vi "example test.vi"() -> (3 "correct execution settings":bool)   [LabVIEW 2015, in "tdms logger tests.lvlib"]
uses:
  tdms logger tests.lvlib
  execution/TDMS datalogger runtime.lvclass
  <vilib>/NI/Tag Bus/dictionary/data dictionary.lvclass/data dictionary.ctl
  <vilib>/NI/Tag Bus/dictionary/lookup polymorphs/locate double.vi
  <vilib>/NI/Tag Bus/table/data polymorphs/write one/write Double.vi
  <vilib>/NI/Tag Bus/dictionary/search/find data index.vi
  <vilib>/NI/Tag Bus/dictionary/search/search string list.vi
  <vilib>/NI/Tag Bus/dictionary/tag not found.vi
  configuration/TDMS datalogger configuration.lvclass
  <vilib>/NI/Tag Bus Module Framework/channel/TBM channel.lvclass
  <vilib>/NI/Tag Bus/tag/Data Type.ctl
  <vilib>/NI/Tag Bus/tag/tag descriptor.lvclass
  <vilib>/NI/Tag Bus Module Framework/channel/channel classification.ctl
  <vilib>/NI/Tag Bus/dictionary/data dictionary.lvclass
  <vilib>/NI/Tag Bus/table/data table.lvlib
  <vilib>/NI/Configuration Framework/serializable configuration/NISE_CEF_serializable configuration.lvclass
panel:
  out "final error":errorcluster
  out "output error":errorcluster
  out "output lookup error":errorcluster
  out "init error":errorcluster
  out "serialization problem":errorcluster
  out "invalid configuration":errorcluster
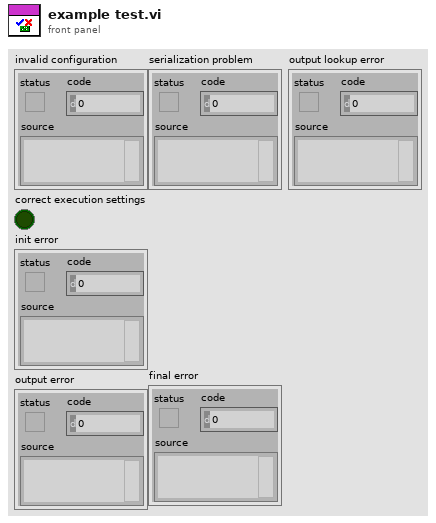
[diagram p1: front panel]
types:
  T1 = typedef "TBM channel.lvclass/channel classification.ctl" = enum16{"input data", "output data", "processing parameter", "processing result"}
  T2 = typedef "tag bus.lvlib/tag descriptor.lvclass/Data Type.ctl" = enum16{"Double", "Single", "I64", "I32", "I16", "I8", "U64", "U32", "U16", "U8", "Boolean", "String", "Array of Double", "Array of Single", "Array of I64", "Array of I32", "Array of I16", "Array of I8", "Array of U64", "Array of U32", "Array of U16", "Array of U8", "Array of Boolean", "Array of String"}
  T3 = typedef "TBM channel.lvclass/data tables.ctl" = cluster{"input data":T4, "processing parameter":T4, "processing result":T4, "output data":T4}
  T4 = typedef "tag bus.lvlib/dictionary table pair.ctl" = cluster{"data dictionary":refnum<class "data dictionary.lvclass">, "data table":T5}
  T5 = typedef "tag bus.lvlib/data table.lvlib/data table.ctl" = cluster{"Double":dbl[], "Single":sgl[], "I64":i64[], "I32":i32[], "I16":i16[], "I8":i8[], "U64":u64[], "U32":u32[], "U16":u16[], "U8":u8[], "Boolean":bool[], "String":string[], "Array of Double":cluster{"DBL Array":dbl[]}[], "Array of Single":cluster{"SGL Array":sgl[]}[], "Array of I64":cluster{"I64 Array":i64[]}[], "Array of I32":cluster{"I32 Array":i32[]}[], "Array of I16":cluster{"I16 Array":i16[]}[], "Array of I8":cluster{"I8 Array":i8[]}[], "Array of U64":cluster{"U64 Array":u64[]}[], "Array of U32":cluster{"U32 Array":u32[]}[], "Array of U16":cluster{"U16 Array":u16[]}[], "Array of U8":cluster{"U8 Array":u8[]}[], "Array of Boolean":cluster{"Boolean Array":bool[]}[], "Array of String":cluster{"String Array":string[]}[]}
  T6 = typedef "TBM module execution interface.lvclass/execution settings.ctl" = cluster{"reads inputs":bool, "processes data":bool, "writes outputs":bool}
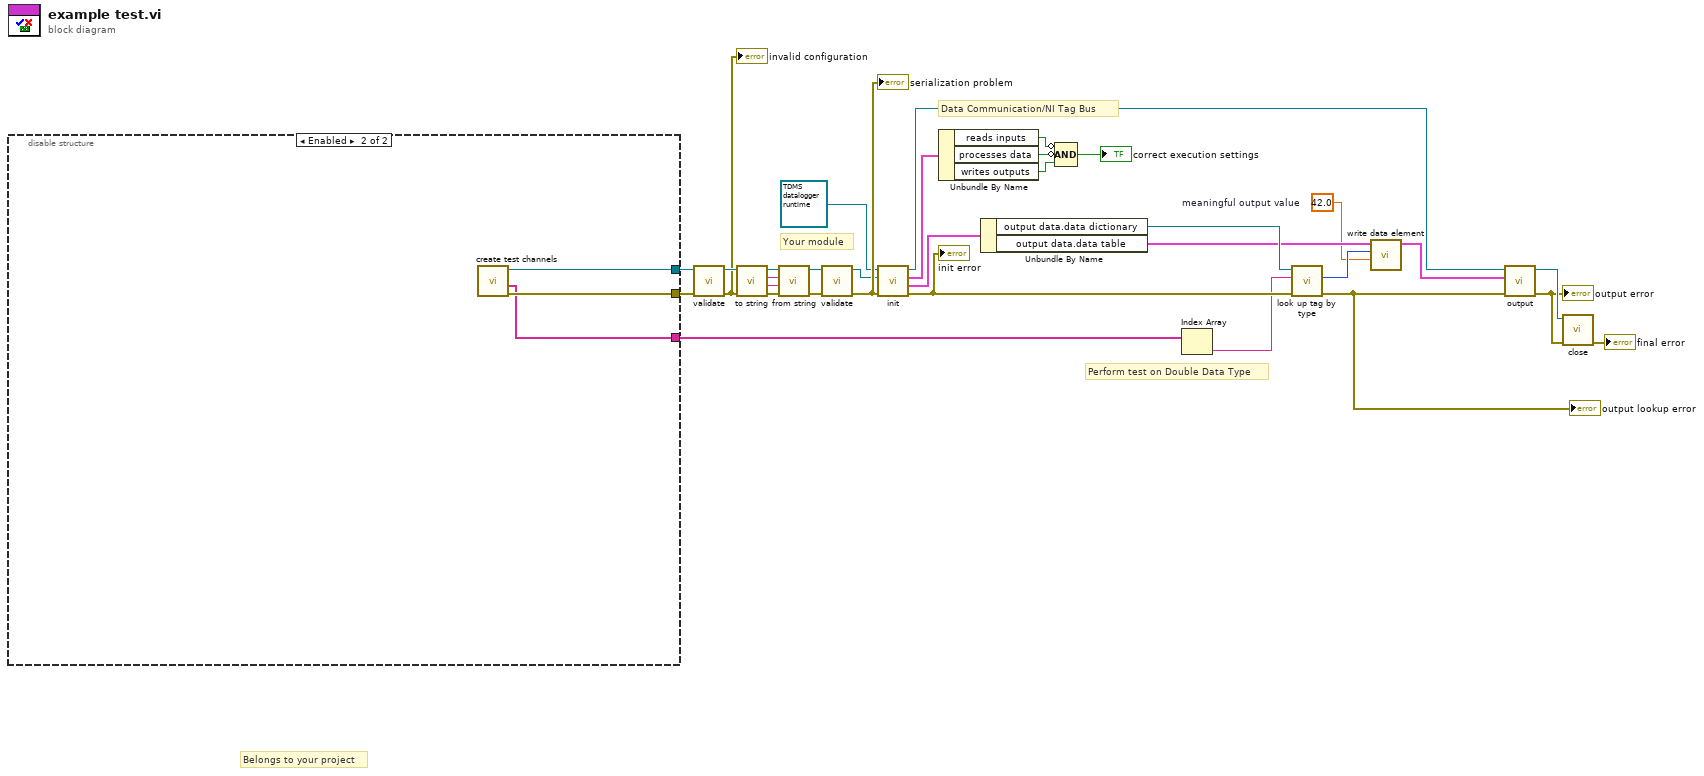
[diagram p0: block diagram]
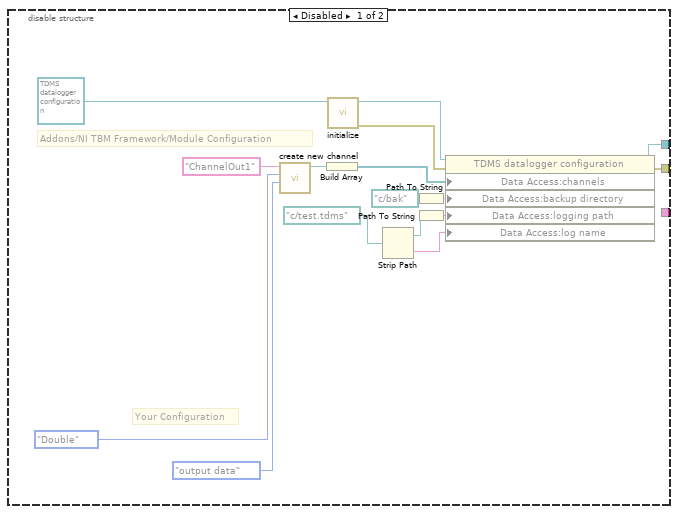
[diagram p2: hidden frame]
diagram:
  w11 = 42.0  # meaningful output value
  # "Perform test on Double Data Type"
  # "Data Communication/NI Tag Bus"
  # "Your module"
  # "Belongs to your project"
  n1 = disable-structure shown="Enabled" {
    disable-tunnel: [w44 w50] -> w5
    disable-tunnel: [w43 w51] -> w4
    disable-tunnel: [_ w49] -> w2
    frame Disabled {
      # "Your Configuration"
      # "Addons/NI TBM Framework/Module Configuration"
      n2 = call <vilib>:"create new channel.vi"("channel classification"=channel_classification."output data", "data type"=Data_Type."Double", "channel name"="ChannelOut1") -> ("channel"=w45:refnum<class "TBM channel.lvclass">)  [unwired: 8 in]
      n3 = Build Array(w45) -> (w42:refnum<class "TBM channel.lvclass">[])
      n4 = call <vilib>:"initialize.vi"("configuration in"=refnum<class "TDMS datalogger configuration.lvclass"> refnum ("TDMS datalogger configuration")) -> ("error out"=w38:errorcluster, "configuration out"=w39:refnum<class "TDMS datalogger configuration.lvclass">)  [unwired: 8 in, 1 out]
      n5 = Strip Path(path=path "c:/test.tdms" ("logging path")) -> (stripped path=w35:path, name=w33:string)
      n6 = Path To String(path=path "c:/bak" ("backup directory")) -> (string=w37:string)
      n7 = Path To String(path=w35) -> (string=w34:string)
      n8 = property class="TDMS datalogger configuration"(reference=w39, error in=w38, "Data Access:channels"=w42, "Data Access:backup directory"=w37, "Data Access:logging path"=w34, "Data Access:log name"=w33) -> (reference out=w44:refnum<class "TDMS datalogger configuration.lvclass">, error out=w43:errorcluster)
    }
    frame Enabled {
      n9 = call "create test channels.vi"() -> ("error out"=w51:errorcluster, "channel names"=w49:string[], "TDMS datalogger configuration out"=w50:refnum<class "TDMS datalogger configuration.lvclass">)  [unwired: 4 in, 5 out]
    }
  }
  n10 = call-dynamic "validate.vi"("error in"=w4, "TDMS datalogger configuration in"=w5) -> ("error out"=w31:errorcluster, "TDMS datalogger configuration out"=w32:refnum<class "TDMS datalogger configuration.lvclass">)  [unwired: 8 in]
  "invalid configuration" <- w31
  n11 = call-dynamic "to string.vi"("error in"=w31, "TDMS datalogger configuration in"=w32) -> ("error out"=w27:errorcluster, "data"=w28:string, "version"=w29:string, "TDMS datalogger configuration out"=w30:refnum<class "TDMS datalogger configuration.lvclass">)  [unwired: 6 in]
  n12 = call-dynamic "from string.vi"("error in"=w27, "data"=w28, "version"=w29, "TDMS datalogger configuration in"=w30) -> ("error out"=w25:errorcluster, "TDMS datalogger configuration out"=w26:refnum<class "TDMS datalogger configuration.lvclass">)  [unwired: 6 in]
  n13 = call-dynamic "validate.vi"("error in"=w25, "TDMS datalogger configuration in"=w26) -> ("error out"=w24:errorcluster, "TDMS datalogger configuration out"=w23:refnum<class "TDMS datalogger configuration.lvclass">)  [unwired: 8 in]
  "serialization problem" <- w24
  n14 = call-dynamic "init.vi"("error in"=w24, "TBM module configuration in"=w23, "TDMS datalogger runtime in"=refnum<class "TDMS datalogger runtime.lvclass"> refnum ("TDMS datalogger runtime")) -> ("error out"=w16:errorcluster, "data allocations"=w17:T3, "execution settings"=w22:T6, "TDMS datalogger runtime out"=w15:refnum<class "TDMS datalogger runtime.lvclass">)  [unwired: 5 in]
  "init error" <- w16
  n15 = Unbundle By Name(w22) -> ("reads inputs"=w19:bool, "processes data"=w21:bool, "writes outputs"=w20:bool)
  n16 = Unbundle By Name(w17) -> ("output data.data dictionary"=w14:refnum<class "data dictionary.lvclass">, "output data.data table"=w12:T5)
  n17 = Compound Arithmetic op=AND(invert w19, invert w21, w20) -> (→"correct execution settings":bool)
  n18 = Index Array(array=w2) -> (element=w1:string)  [unwired: 1 in]
  n19 = call-poly <vilib>:"look up tag by type.vi"("error in"=w16, "name"=w1, "data dictionary in"=w14) -> ("error out"=w10:errorcluster, "index"=w13:i32)  [unwired: 6 in, 1 out]
  "output lookup error" <- w10
  n20 = call-poly <vilib>:"write data element.vi"("value"=w11, "index"=w13, "data table in"=w12) -> ("data table out"=w9:T5)  [unwired: 8 in]
  n21 = call-dynamic "output.vi"("error in"=w10, "data table in"=w9, "TDMS datalogger runtime in"=w15) -> ("error out"=w7:errorcluster, "TDMS datalogger runtime out"=w8:refnum<class "TDMS datalogger runtime.lvclass">)  [unwired: 6 in, 1 out]
  "output error" <- w7
  n22 = call-dynamic "close.vi"("error in"=w7, "TDMS datalogger runtime in"=w8) -> ("error out"=→"final error":errorcluster)  [unwired: 9 in]
